vi "LabApp - Tag List Editor for Data Viewer.vi"(7 "Default":string, 9 "Tag List in":string[](array[string])) -> (0 "cancel out":bool, 3 "Tag List out":string[](array[string]))   [LabVIEW 2021]
doc: "::: CalcExpress Toolkit :::\nCopyright (c) 2000-2026 Konstantin Shifershteyn. All rights reserved."
panel:
  in  "default":bool
  in  "cancel":bool
  in  "ok":bool
  in  "Tag List":string
  # "[1] Type tag names in separate lines.\n[2] Note that a tag is an alias associated with a variable.\n    The target variable may belong to any application\n    that uses VarMan to maintain variables."
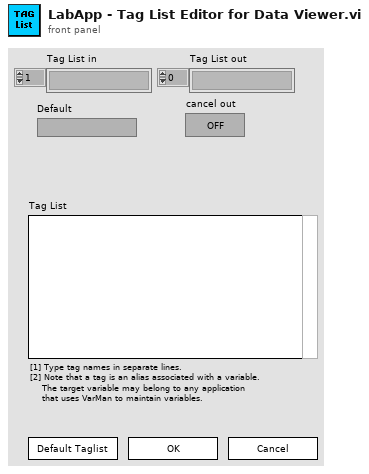
[diagram p1: front panel]
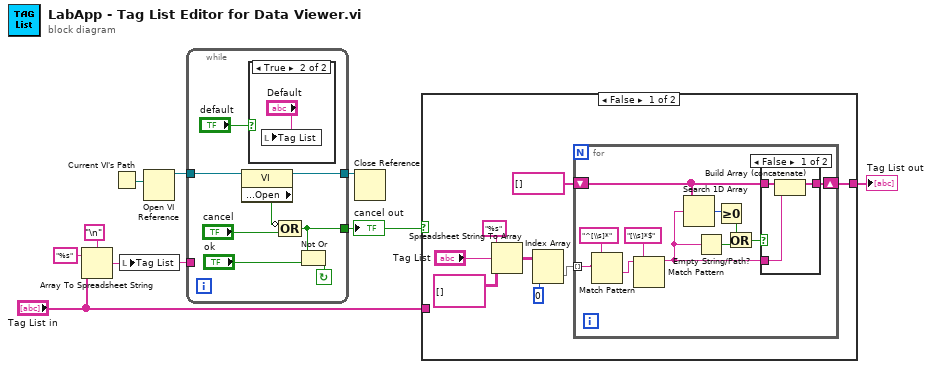
[diagram p0: block diagram]
diagram:
  n1 = Array To Spreadsheet String(delimiter (Tab)="\n", array="Tag List in", 3:"%s" ("format string")) -> (spreadsheet string=w4:string)
  n2 = Current VI's Path() -> (path=w7:path)
  n3 = local write "Tag List"(w4) -> ()
  n4 = Open VI Reference(vi path=w7) -> (vi reference=w9:refnum<vi>)  [unwired: 5 in, 1 out]
  n5 = while {
    tunnel: w4 -> [_]
    tunnel: [w11] -> w8
    tunnel: [w12] -> w3
    tunnel: w9 -> [w17]
    stop <- w13 continue-if-true
    n6 = property class="VI"(reference=w17) -> (reference out=w11:refnum<vi>, "Front Panel Window:Open"=w15:bool)  [unwired: 1 in, 1 out]
    n7 = case shown="True" "default" {
      frame False {
      }
      frame True {
        n8 = local write "Tag List"("Default") -> ()
      }
    }
    n9 = Compound Arithmetic op=OR(invert w15, "cancel") -> (w12:bool)
    n10 = Not Or(1:"ok", 2:w12) -> (0:w13:bool)
  }
  "cancel out" <- w3
  n11 = Close Reference(reference=w8) -> ()  [unwired: 1 in, 1 out]
  n12 = case shown="False" w3 {
    tunnel: [w19 w42] -> w2
    tunnel: "Tag List in" -> [_ w42]
    frame False {
      n13 = Spreadsheet String To Array(format string="%s", spreadsheet string="Tag List", array type (2D Dbl)=string[][] []) -> (array=w23:string[][])  [unwired: 1 in]
      n14 = Index Array(array=w23, index (col)=0) -> (element=w21:string[])  [unwired: 1 in]
      n15 = for {
        tunnel: w21 -> [w37] mode=indexing
        shift-right: [w28] -> w19
        shift-left: string[] [] -> [w29]
        n16 = Match Pattern(string=w37, regular expression="^[\\s]*") -> (after substring=w35:string)  [unwired: 1 in, 3 out]
        n17 = Match Pattern(string=w35, regular expression="[\\s]*$") -> (before substring=w27:string)  [unwired: 1 in, 3 out]
        n18 = Search 1D Array(1D array=w29, element=w27) -> (index of element=w31:i32)  [unwired: 1 in]
        n19 = Empty String/Path?(string/path=w27) -> (empty?=w33:bool)
        n20 = Greater Or Equal To 0?(x=w31) -> (x >= 0?=w32:bool)
        n21 = Or(x=w32, y=w33) -> (x .or. y?=w30:bool)
        n22 = case shown="False" w30 {
          tunnel: w29 -> [w40 w41]
          tunnel: [w39 w41] -> w28
          tunnel: w27 -> [w38 _]
          frame False {
            n23 = Build Array (concatenate)(w40, w38) -> (w39:string[])
          }
          frame True {
          }
        }
      }
    }
    frame True {
    }
  }
  "Tag List out" <- w2
